vi "Measurement Logic.vi"(8 "error in":errorcluster, 9 "measurement configuration":T2={"Automation Test"=FALSE, "Power sequencing file path"="", "RFmxVNA name"="5842_0", "vCal Name"="VNA-5633", "RFmxVNA Calset Enable"=FALSE, "RFmxVNA Calset Interpolation"=FALSE, "Calset File Path (String)"="", "RFmxVNA attenuation mode"=enum."s2p File", "RFmxVNA Port1 s2p file path (String)"="", "RFmxVNA Port1 s-parameters orientation"=enum."Port2 Towards DUT", "RFmxVNA Port1 Power Compensation"=FALSE, "RFmxVNA Port2 s2p file path (String)"="", "RFmxVNA Port2 s-parameters orientation"=enum."Port1 Towards DUT", "RFmxVNA Port2 Power Compensation"=FALSE, "Port1 Power Level (dBm)"=2.0, "Port1 Test Receiver Attenuation (dB)"=1.2, "Port2 Power Level (dBm)"=2.0, "Port2 Test Receiver Attenuation (dB)"=1.2, "IF Bandwidth (Hz)"=1.0, "Action"=enum."Measure", "Pulse Mode Enabled"=FALSE, "Pulse Period"=0.001, "Pulse Modulator Delay"=0.0, "Pulse Modulator Width"=0.0001, "Pulse Acquisition Auto"=FALSE, "Pulse Acquisition Delay"=2e-05, "Pulse Acquisition Width"=4.665e-05, "Start Frequency (Hz)"=4000000000.0, "Stop Frequency (Hz)"=26000000000.0, "Number of Points"=200, "Measurement S-Parameters"=["S11", "S12", "S21", "S22"], "Phase Trace Type"=0, "Magnitude Units"=0, "SnP File Path (String)"="", "Averaging Enabled"=FALSE, "Averaging Count"=0, "Power sequencing file validity check"=TRUE} {"Magnitude Units" items=["dB", "Linear"]; "Phase Trace Type" items=["Wrapped", "Unwrapped"]; "Stop Frequency (Hz)" format="%.3p"; "Start Frequency (Hz)" format="%.3p"; "Pulse Acquisition Width" format="%.2p"; "Pulse Acquisition Delay" format="%.2p"; "Pulse Modulator Width" format="%.2p"; "Pulse Modulator Delay" format="%.2p"; "Pulse Period" format="%.2p"; "IF Bandwidth (Hz)" format="%.2p"; "Port2 Test Receiver Attenuation (dB)" format="%.2f"; "Port2 Power Level (dBm)" format="%.2f"; "Port1 Test Receiver Attenuation (dB)" format="%.2f"; "Port1 Power Level (dBm)" format="%.2f"}, 10 "measure call context in":refnum<class "Measure Call Context.lvclass">) -> (0 "error out":errorcluster, 1 "measurement results":T1, 2 "measure call context out":refnum<class "Measure Call Context.lvclass">)   [LabVIEW 2023, in "FPT_SParam.lvclass"]
doc: "Contains the core logic for executing the measurement."
uses:
  FPT_SParam.lvclass
  FPT_SParam.lvclass/FPT_SParam.ctl
  Measurement Configuration.ctl
  Measurement Results.ctl
  <vilib>/Analysis/NI_AALBase.lvlib
  <vilib>/Analysis/baseanly.llb/Mean (DBL).vi
  <vilib>/Plug-In SDKs/Measurements/Measure Call Context/Measure Call Context.lvclass
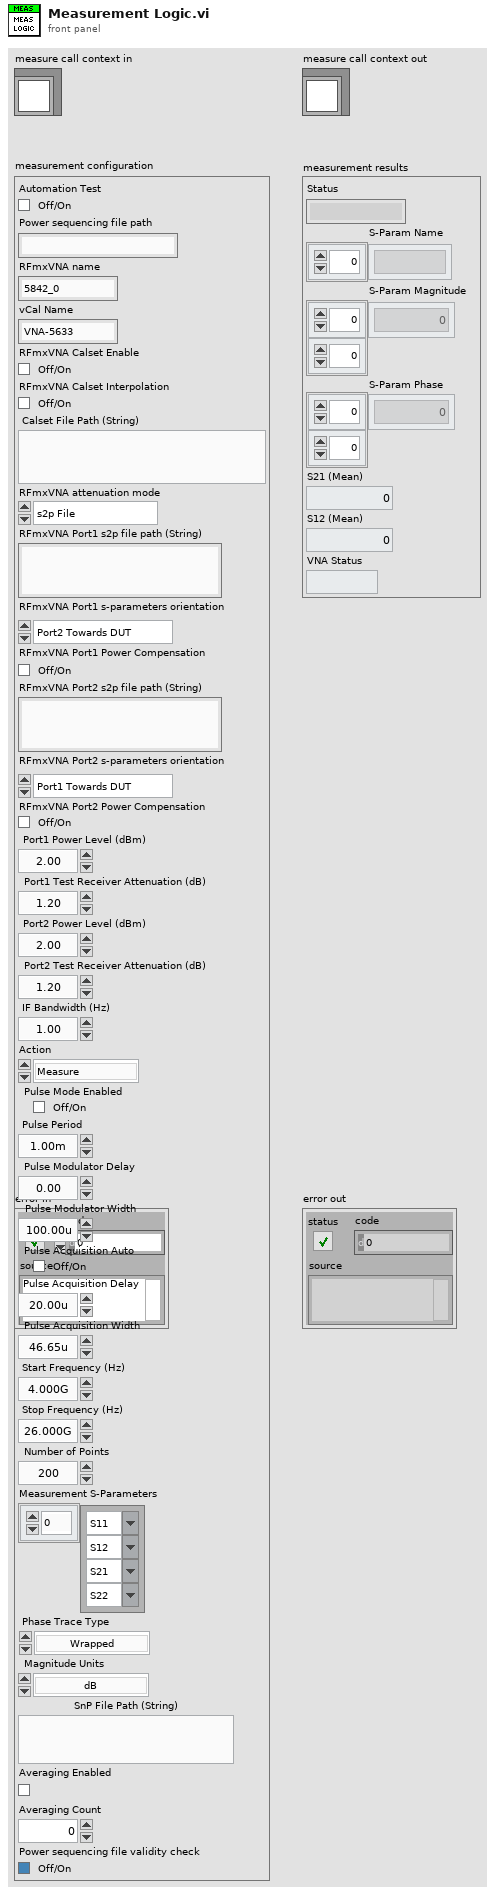
[diagram p1: front panel]
types:
  T1 = typedef "FPT_SParam.lvclass/Measurement Results.ctl" = cluster{"Status":string, "S-Param Name":string[], "S-Param Magnitude":dbl[][], "S-Param Phase":dbl[][], "S21 (Mean)":dbl, "S12 (Mean)":dbl, "VNA Status":string}
  T2 = typedef "FPT_SParam.lvclass/Measurement Configuration.ctl" = cluster{"Automation Test":bool, "Power sequencing file path":string, "RFmxVNA name":string, "vCal Name":string, "RFmxVNA Calset Enable":bool, "RFmxVNA Calset Interpolation":bool, "Calset File Path (String)":string, "RFmxVNA attenuation mode":enum32{"<None>", "s2p File"}, "RFmxVNA Port1 s2p file path (String)":string, "RFmxVNA Port1 s-parameters orientation":enum32{"Port1 Towards DUT", "Port2 Towards DUT"}, "RFmxVNA Port1 Power Compensation":bool, "RFmxVNA Port2 s2p file path (String)":string, "RFmxVNA Port2 s-parameters orientation":enum32{"Port1 Towards DUT", "Port2 Towards DUT"}, "RFmxVNA Port2 Power Compensation":bool, "Port1 Power Level (dBm)":dbl, "Port1 Test Receiver Attenuation (dB)":dbl, "Port2 Power Level (dBm)":dbl, "Port2 Test Receiver Attenuation (dB)":dbl, "IF Bandwidth (Hz)":dbl, "Action":enum32{"Calibrate", "Measure"}, "Pulse Mode Enabled":bool, "Pulse Period":dbl, "Pulse Modulator Delay":dbl, "Pulse Modulator Width":dbl, "Pulse Acquisition Auto":bool, "Pulse Acquisition Delay":dbl, "Pulse Acquisition Width":dbl, "Start Frequency (Hz)":dbl, "Stop Frequency (Hz)":dbl, "Number of Points":i32, "Measurement S-Parameters":string[], "Phase Trace Type":i32, "Magnitude Units":i32, "SnP File Path (String)":string, "Averaging Enabled":bool, "Averaging Count":u32, "Power sequencing file validity check":bool}
  T3 = cluster{"measurement configuration":T2, "measurement results":T1, "CustomData":cluster{"Valid CSV":bool}}
  T4 = enum32{"Power On Dut", "Switching", "De-embedding + Measurement", "Power Off Dut"}[]
  T5 = typedef "RFmxVNA Config - SParam.ctl" = cluster{"Resource Name":refnum<k15>, "vCal Name":string, "RFmxVNA Calset Enable":bool, "RFmxVNA Calset Interpolation":bool, "Calset File Path":string, "RFmxVNA attenuation mode":enum32{"<None>", "s2p File"}, "RFmxVNA Port1 s2p file path":string, "RFmxVNA Port1 s-parameters orientation":enum32{"Port1 Towards DUT", "Port2 Towards DUT"}, "RFmxVNA Port1 Power Compensation":bool, "RFmxVNA Port2 s2p file path":string, "RFmxVNA Port2 s-parameters orientation":enum32{"Port1 Towards DUT", "Port2 Towards DUT"}, "RFmxVNA Port2 Power Compensation":bool, "Port1 Power Level (dBm)":dbl, "Port1 Test Receiver Attenuation (dB)":dbl, "Port2 Power Level (dBm)":dbl, "Port2 Test Receiver Attenuation (dB)":dbl, "IF Bandwidth (Hz)":dbl, "Frequency Sweep":cluster{"Start Frequency (Hz)":dbl, "Stop Frequency (Hz)":dbl, "Number of Points":i32}}
  T6 = typedef "Test Config - SParam.ctl" = cluster{"Action":enum16{"Calibrate", "Measure"}, "Pulse Mode":cluster{"Pulse Mode Enabled":bool, "Pulse Period (s)":dbl, "Pulse Modulator Delay (s)":dbl, "Pulse Modulator Width (s)":dbl, "Pulse Acquisition Auto":bool, "Pulse Acquisition Delay (s)":dbl, "Pulse Acquisition Width (s)":dbl}, "Frequency Sweep":cluster{"Start Frequency (Hz)":dbl, "Stop Frequency (Hz)":dbl, "Number of Points":i32}, "S-Parameters":string[], "Magnitude Units":i32, "Phase Trace Type":i32, "SnP File Path":string, "Averaging Enabled":bool, "Averaging Count":u32}
  T7 = typedef "Event Messenger-bool.lvlib/))Channel.ctl" = refnum<queue>
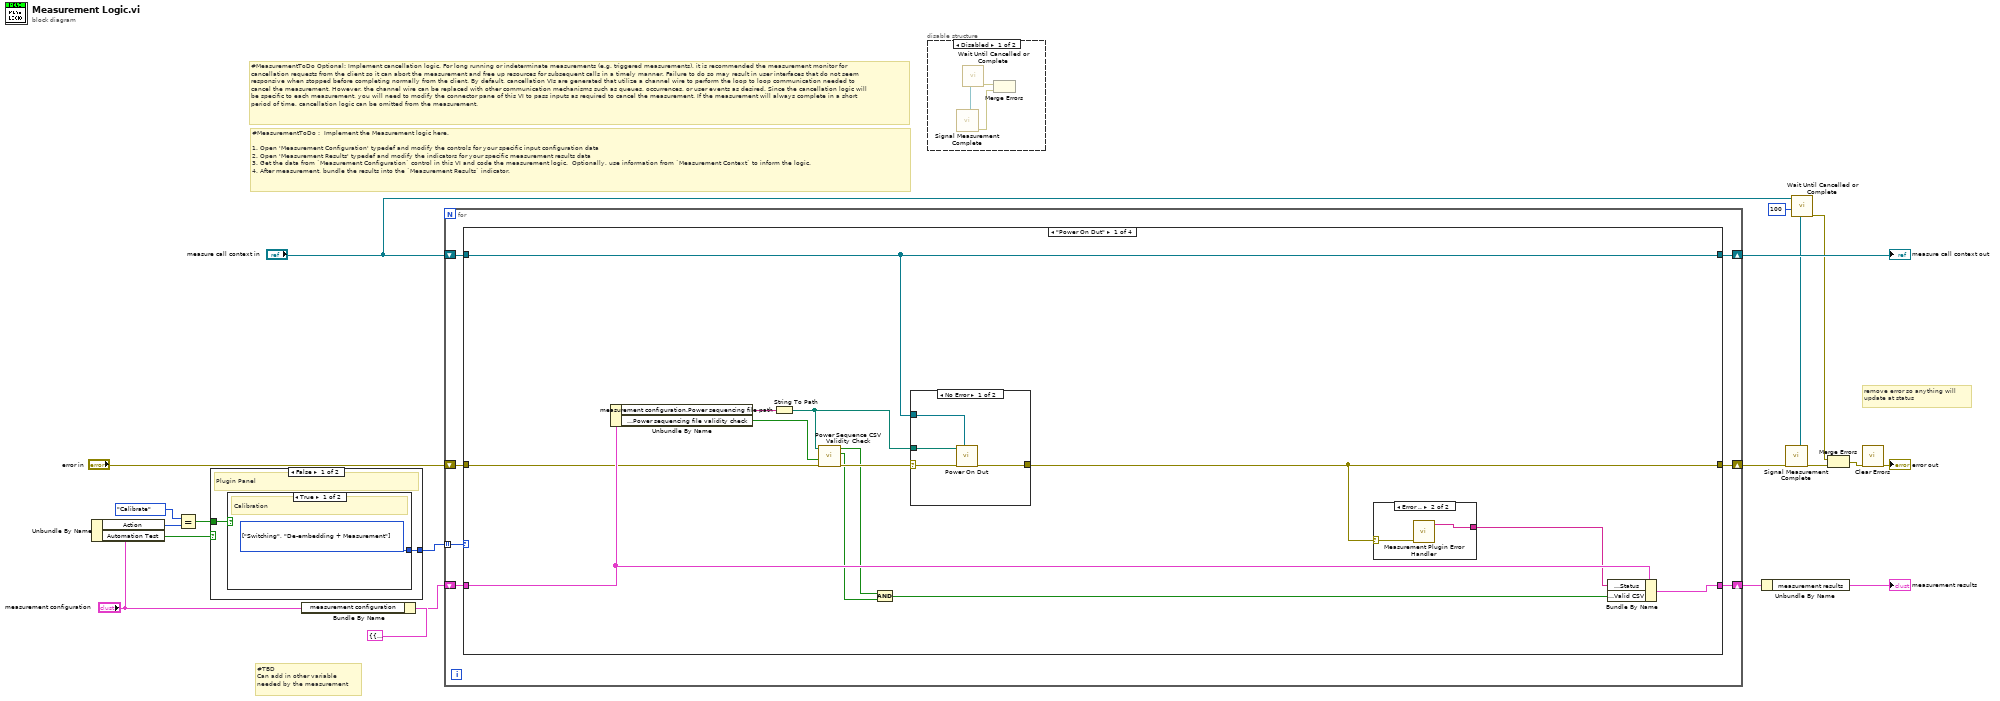
[diagram p0: block diagram]
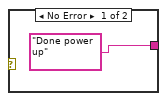
[diagram p3: hidden frame]
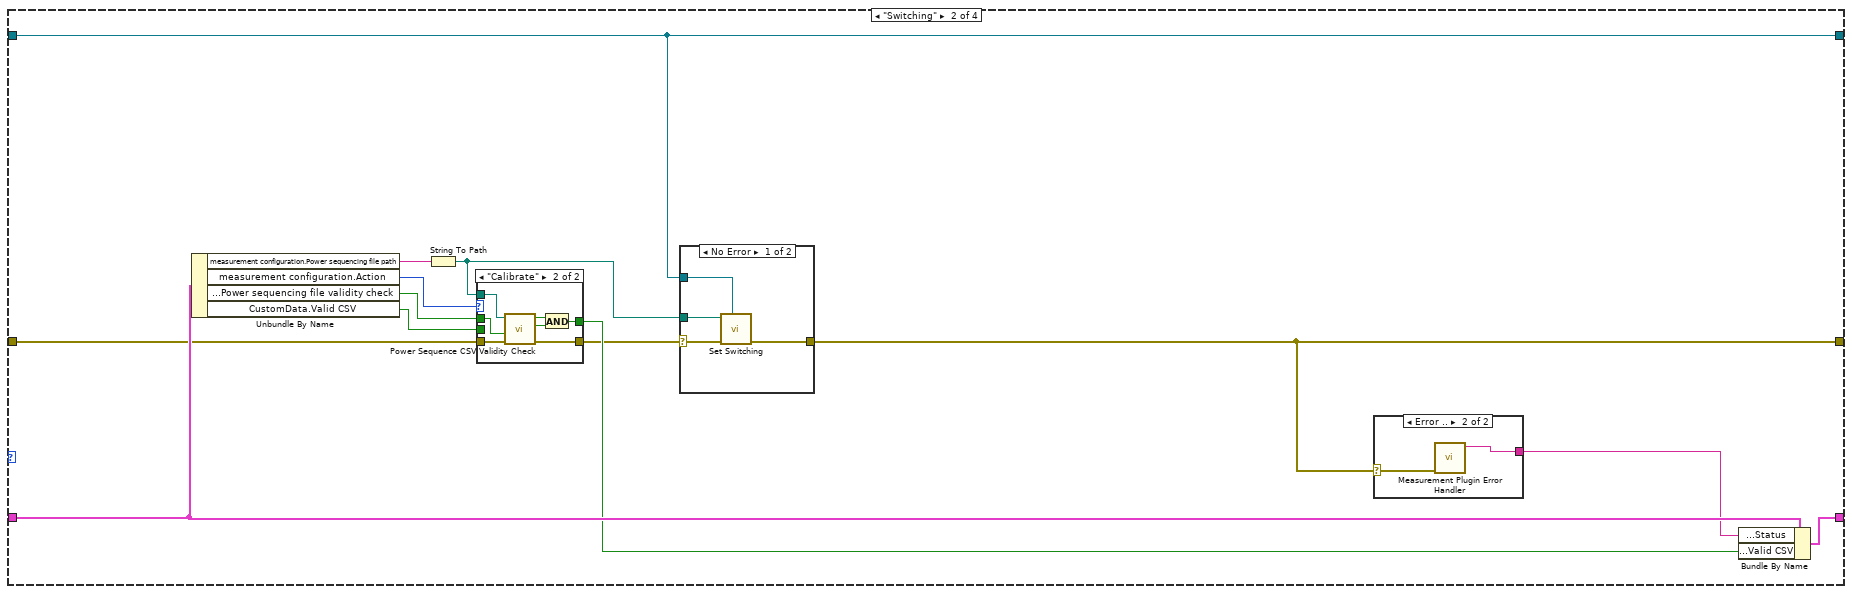
[diagram p4: hidden frame]
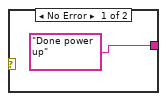
[diagram p7: hidden frame]
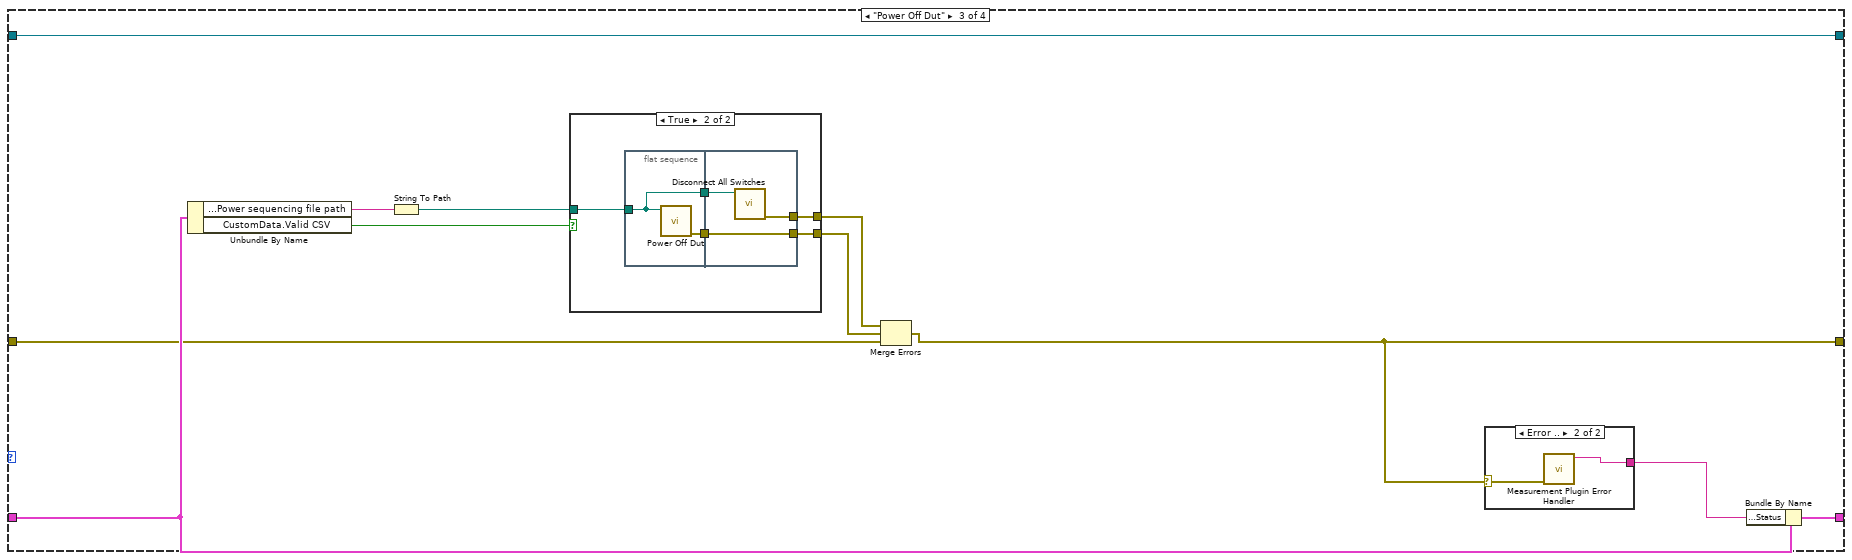
[diagram p8: hidden frame]
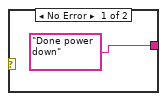
[diagram p10: hidden frame]
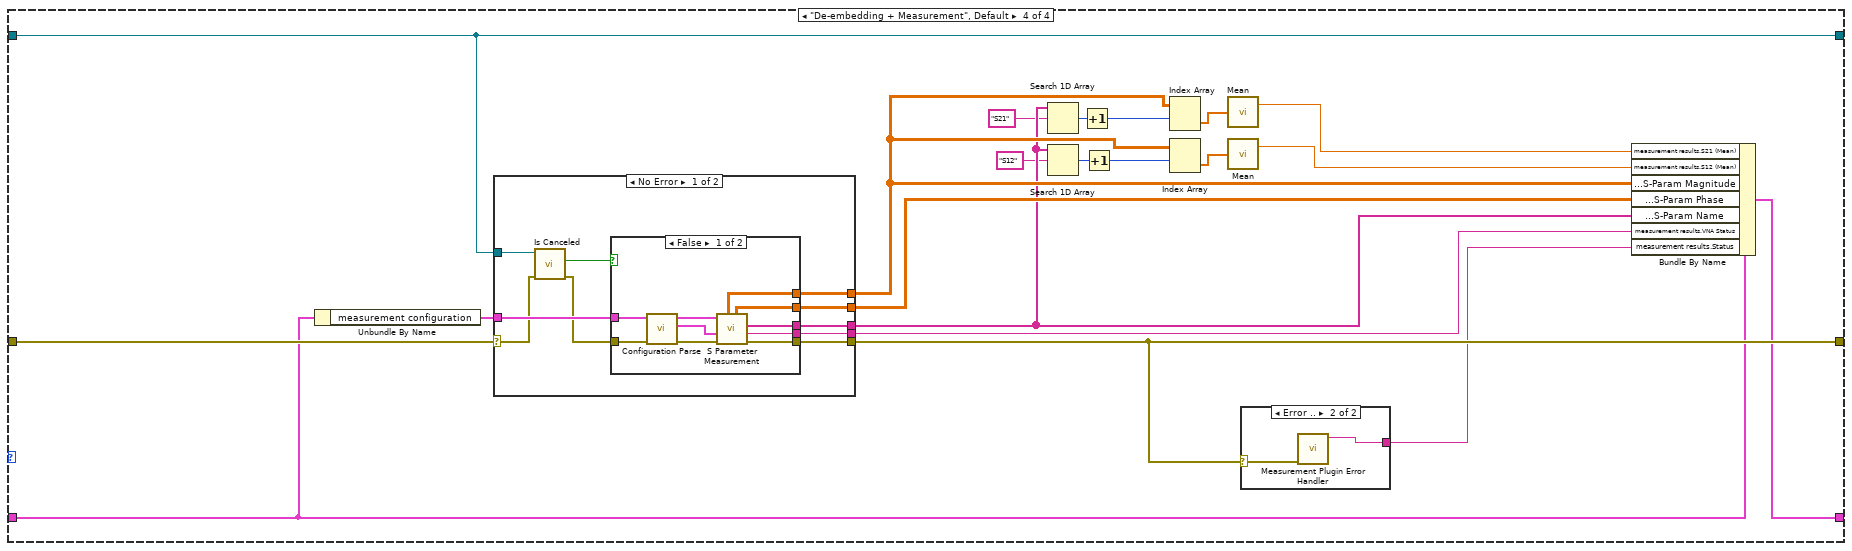
[diagram p11: hidden frame]
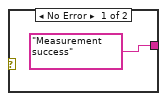
[diagram p12: hidden frame]
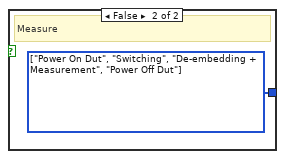
[diagram p16: hidden frame]
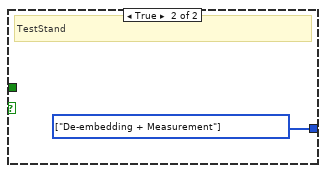
[diagram p17: hidden frame]
diagram:
  # "remove error so anything will\nupdate at status"
  # "#TBD\nCan add in other variable\nneeded by the measurement"
  # "#MeasurementToDo Optional: Implement cancellation logic. For long running or indeterminate measurements (e.g. triggered measurements), it is recommended the measurement monitor for cancellation requests from the client so it can abort the measurement and free up resources for subsequent calls in a timely manner. Failure to do so may result in user interfaces that do not seem responsive when stopped before completing normally from the client. By default, cancellation VIs are generated that utilize a channel wire to perform the loop to loop communication needed to cancel the measurement. However, the channel wire can be replaced with other communication mechanisms such as queues, occurrences, or user events as desired. Since the cancellation logic will be specific to each measurement, you will need to modify the connector pane of this VI to pass inputs as required to cancel the measurement. If the measurement will always complete in a short period of time, cancellation logic can be omitted from the measurement."
  # "#MeasurementToDo :  Implement the Measurement logic here.\n\n1. Open 'Measurement Configuration' typedef and modify the controls for your specific input configuration data\n2. Open 'Measurement Results' typedef and modify the indicators for your specific measurement results data\n3. Get the data from `Measurement Configuration` control in this VI and code the measurement logic.  Optionally, use information from `Measurement Context` to inform the logic.\n4. After measurement, bundle the results into the `Measurement Results` indicator."
  n1 = Unbundle By Name("measurement configuration") -> ("Action"=w12:enum32{"Calibrate", "Measure"}, "Automation Test"=w9:bool)
  n2 = Equal?(x=enum32{"Calibrate", "Measure"}."Calibrate", y=w12) -> (x = y?=w8:bool)
  n3 = case shown="False" w9 {
    tunnel: [w22 w25] -> w10
    tunnel: w8 -> [w21 _]
    frame False {
      # "Plugin Panel"
      n4 = case shown="True" w21 {
        tunnel: [w23 w24] -> w22
        frame True {
          w23 = T4 [enum."Switching", enum."De-embedding + Measurement"] items=["Power On Dut", "Switching", "De-embedding + Measurement", "Power Off Dut"]
          # "Calibration"
        }
        frame False {
          w24 = T4 [enum."Power On Dut", enum."Switching", enum."De-embedding + Measurement", enum."Power Off Dut"] items=["Power On Dut", "Switching", "De-embedding + Measurement", "Power Off Dut"]
          # "Measure"
        }
      }
    }
    frame True {
      w25 = T4 [enum."De-embedding + Measurement"] items=["Power On Dut", "Switching", "De-embedding + Measurement", "Power Off Dut"]
      # "TestStand"
    }
  }
  n5 = Bundle By Name(cluster=T3 {"measurement configuration"={"Automation Test"=FALSE, "Power sequencing file path"="", "RFmxVNA name"="5842_0", "vCal Name"="VNA-5633", "RFmxVNA Calset Enable"=FALSE, "RFmxVNA Calset Interpolation"=FALSE, "Calset File Path (String)"="", "RFmxVNA attenuation mode"=enum."s2p File", "RFmxVNA Port1 s2p file path (String)"="", "RFmxVNA Port1 s-parameters orientation"=enum."Port2 Towards DUT", "RFmxVNA Port1 Power Compensation"=FALSE, "RFmxVNA Port2 s2p file path (String)"="", "RFmxVNA Port2 s-parameters orientation"=enum."Port1 Towards DUT", "RFmxVNA Port2 Power Compensation"=FALSE, "Port1 Power Level (dBm)"=2.0, "Port1 Test Receiver Attenuation (dB)"=1.2, "Port2 Power Level (dBm)"=2.0, "Port2 Test Receiver Attenuation (dB)"=1.2, "IF Bandwidth (Hz)"=1.0, "Action"=enum."Measure", "Pulse Mode Enabled"=FALSE, "Pulse Period"=0.001, "Pulse Modulator Delay"=0.0, "Pulse Modulator Width"=0.0001, "Pulse Acquisition Auto"=FALSE, "Pulse Acquisition Delay"=2e-05, "Pulse Acquisition Width"=4.665e-05, "Start Frequency (Hz)"=4000000000.0, "Stop Frequency (Hz)"=26000000000.0, "Number of Points"=200, "Measurement S-Parameters"=["S11", "S12", "S21", "S22"], "Phase Trace Type"=0, "Magnitude Units"=0, "SnP File Path (String)"="", "Averaging Enabled"=FALSE, "Averaging Count"=0, "Power sequencing file validity check"=TRUE}, "measurement results"={"Status"="", "S-Param Name"=[], "S-Param Magnitude"=[], "S-Param Phase"=[], "S21 (Mean)"=0.0, "S12 (Mean)"=0.0, "VNA Status"=""}, "CustomData"={"Valid CSV"=FALSE}}, "measurement configuration"="measurement configuration") -> (w18:T3)
  n6 = for {
    tunnel: w10 -> [w31] mode=indexing
    shift-right: [w26] -> w4
    shift-left: "error in" -> [w32]
    shift-right: [w27] -> w16
    shift-left: w18 -> [w30]
    shift-right: [w28] -> w17
    shift-left: "measure call context in" -> [w29]
    n7 = case shown="\"Power On Dut\"" w31 {
      tunnel: w32 -> [w39 w59 w89 w123]
      tunnel: w30 -> [w45 w66 w90 w122]
      tunnel: w29 -> [w40 w61 w93 w109]
      tunnel: [w41 w62 w88 w128] -> w26
      tunnel: [w40 w61 w93 w109] -> w28
      tunnel: [w43 w64 w91 w126] -> w27
      frame "Power On Dut" {
        n8 = Unbundle By Name(w45) -> ("measurement configuration.Power sequencing file path"=w42:string, "measurement configuration.Power sequencing file validity check"=w38:bool)
        n9 = String To Path(string=w42) -> (path=w37:path)
        n10 = call "Power Sequence CSV Validity Check.vi"("error in"=w39, "Enable Validity Check?"=w38, "File Path"=w37) -> ("error out"=w36:errorcluster, "Valid Execution Order"=w34:bool, "All Instruments Available"=w35:bool)  [unwired: 5 in, 1 out]
        n11 = And(x=w35, y=w34) -> (x .and. y?=w33:bool)
        n12 = case shown="No Error" w36 {
          selector: w36 -> [w46 w50]
          tunnel: w37 -> [w49 _]
          tunnel: [w48 w50] -> w41
          tunnel: w40 -> [w47 _]
          frame No Error {
            n13 = call "Power On Dut.vi"("measure call context in"=w47, "error in"=w46, "Power sequencing file path"=w49) -> ("error out"=w48:errorcluster)  [unwired: 7 in, 1 out]
          }
          frame Error {
          }
        }
        n14 = case shown="Error .." w41 {
          selector: w41 -> [_ w53]
          tunnel: ["Done power up" w52] -> w44
          frame No Error {
          }
          frame Error {
            n15 = call "Measurement Plugin Error Handler.vi"("error in"=w53) -> ("Status Message (Error)"=w52:string)  [unwired: 9 in, 1 out]
          }
        }
        n16 = Bundle By Name(cluster=w45, "measurement results.Status"=w44, "CustomData.Valid CSV"=w33) -> (w43:T3)
      }
      frame "Switching" {
        n17 = Unbundle By Name(w66) -> ("measurement configuration.Power sequencing file path"=w63:string, "measurement configuration.Action"=w60:enum32{"Calibrate", "Measure"}, "measurement configuration.Power sequencing file validity check"=w57:bool, "CustomData.Valid CSV"=w56:bool)
        n18 = String To Path(string=w63) -> (path=w58:path)
        n19 = case shown="\"Calibrate\"" w60 {
          tunnel: w59 -> [w68 w75]
          tunnel: [w68 w74] -> w54
          tunnel: [w67 w71] -> w55
          tunnel: w58 -> [_ w70]
          tunnel: w57 -> [_ w69]
          tunnel: w56 -> [w67 _]
          frame Default {
          }
          frame "Calibrate" {
            n20 = call "Power Sequence CSV Validity Check.vi"("error in"=w75, "Enable Validity Check?"=w69, "File Path"=w70) -> ("error out"=w74:errorcluster, "Valid Execution Order"=w72:bool, "All Instruments Available"=w73:bool)  [unwired: 5 in, 1 out]
            n21 = And(x=w73, y=w72) -> (x .and. y?=w71:bool)
          }
        }
        n22 = case shown="No Error" w54 {
          selector: w54 -> [w76 w80]
          tunnel: [w79 w80] -> w62
          tunnel: w58 -> [w78 _]
          tunnel: w61 -> [w77 _]
          frame No Error {
            n23 = call "Set Switching.vi"("measure call context in"=w77, "error in"=w76, "File Path"=w78) -> ("error out"=w79:errorcluster)  [unwired: 7 in, 1 out]
          }
          frame Error {
          }
        }
        n24 = case shown="Error .." w62 {
          selector: w62 -> [_ w83]
          tunnel: ["Done power up" w82] -> w65
          frame No Error {
          }
          frame Error {
            n25 = call "Measurement Plugin Error Handler.vi"("error in"=w83) -> ("Status Message (Error)"=w82:string)  [unwired: 9 in, 1 out]
          }
        }
        n26 = Bundle By Name(cluster=w66, "measurement results.Status"=w65, "CustomData.Valid CSV"=w55) -> (w64:T3)
      }
      frame "Power Off Dut" {
        n27 = Unbundle By Name(w90) -> ("measurement configuration.Power sequencing file path"=w94:string, "CustomData.Valid CSV"=w84:bool)
        n28 = String To Path(string=w94) -> (path=w87:path)
        n29 = case shown="True" w84 {
          tunnel: w87 -> [_ w97]
          tunnel: [_ w96] -> w86
          tunnel: [_ w95] -> w85
          frame False {
          }
          frame True {
            n30 = flat-sequence {
              tunnel: w97 -> [w100]
              tunnel: [w101] -> w99
              tunnel: [w100] -> w98
              tunnel: [w104] -> w96
              tunnel: w99 -> [w104]
              tunnel: [w103] -> w95
              tunnel: w98 -> [w102]
              frame #0 {
                n31 = call "Power Off Dut.vi"("Power Sequencing File Path"=w100) -> ("error out"=w101:errorcluster)  [unwired: 10 in]
              }
              frame #1 {
                n32 = call "Disconnect All Switches.vi"("File Path"=w102) -> ("error out"=w103:errorcluster)  [unwired: 10 in]
              }
            }
          }
        }
        n33 = Merge Errors(w85, w86, w89) -> (w88:errorcluster)
        n34 = case shown="Error .." w88 {
          selector: w88 -> [_ w107]
          tunnel: ["Done power down" w106] -> w92
          frame No Error {
          }
          frame Error {
            n35 = call "Measurement Plugin Error Handler.vi"("error in"=w107) -> ("Status Message (Error)"=w106:string)  [unwired: 9 in, 1 out]
          }
        }
        n36 = Bundle By Name(cluster=w90, "measurement results.Status"=w92) -> (w91:T3)
      }
      frame "De-embedding + Measurement", Default {
        n37 = Unbundle By Name(w122) -> ("measurement configuration"=w108:T2)
        n38 = case shown="No Error" w123 {
          selector: w123 -> [w135 w153]
          tunnel: [w141 w153] -> w128
          tunnel: [w140 _] -> w117
          tunnel: [w139 _] -> w125
          tunnel: [w138 _] -> w124
          tunnel: [w137 _] -> w116
          tunnel: w108 -> [w136 _]
          tunnel: w109 -> [w132 _]
          frame No Error {
            n39 = call <vilib>:"Is Canceled.vi"("error in"=w135, "measure call context in"=w132) -> ("error out"=w134:errorcluster, "is canceled?"=w133:bool)  [unwired: 7 in, 1 out]
            n40 = case shown="False" w133 {
              tunnel: [w151 w152] -> w141
              tunnel: [w147 _] -> w140
              tunnel: [w146 _] -> w139
              tunnel: [w145 _] -> w138
              tunnel: [w144 _] -> w137
              tunnel: w136 -> [w143 _]
              tunnel: w134 -> [w142 w152]
              frame False {
                n41 = call "Configuration Parse.vi"("error in"=w142, "Measurement Configuration"=w143) -> ("error out"=w149:errorcluster, "RFmxVNA Settings"=w150:T5, "Test Configuration"=w148:T6)  [unwired: 7 in]
                n42 = call "S Parameter Measurement.vi"("error in"=w149, "RFmxVNA Settings"=w150, "Test Configuration"=w148) -> ("error out"=w151:errorcluster, "VNA Status"=w145:string, "S-Param Name"=w144:string[], "S-Param Phase"=w146:dbl[][], "S-Param Magnitude"=w147:dbl[][])  [unwired: 3 in, 1 out]
              }
              frame True {
              }
            }
          }
          frame Error {
          }
        }
        n43 = Search 1D Array(1D array=w116, element="S21") -> (index of element=w113:i32)  [unwired: 1 in]
        n44 = Search 1D Array(1D array=w116, element="S12") -> (index of element=w111:i32)  [unwired: 1 in]
        n45 = Increment(x=w113) -> (x+1=w112:i32)
        n46 = Increment(x=w111) -> (x+1=w110:i32)
        n47 = Index Array(array=w117, index (row)=w112) -> (element=w121:dbl[])  [unwired: 1 in]
        n48 = Index Array(array=w117, index (row)=w110) -> (element=w119:dbl[])  [unwired: 1 in]
        n49 = call-poly <vilib>:"Mean.vi"("X"=w121) -> ("mean"=w120:dbl)  [unwired: 1 out]
        n50 = call-poly <vilib>:"Mean.vi"("X"=w119) -> ("mean"=w118:dbl)  [unwired: 1 out]
        n51 = case shown="Error .." w128 {
          selector: w128 -> [_ w131]
          tunnel: ["Measurement success" w130] -> w127
          frame No Error {
          }
          frame Error {
            n52 = call "Measurement Plugin Error Handler.vi"("error in"=w131) -> ("Status Message (Error)"=w130:string)  [unwired: 9 in, 1 out]
          }
        }
        n53 = Bundle By Name(cluster=w122, "measurement results.S21 (Mean)"=w120, "measurement results.S12 (Mean)"=w118, "measurement results.S-Param Magnitude"=w117, "measurement results.S-Param Phase"=w125, "measurement results.S-Param Name"=w116, "measurement results.VNA Status"=w124, "measurement results.Status"=w127) -> (w126:T3)
      }
    }
  }
  "measure call context out" <- w17
  n54 = disable-structure shown="Disabled" {
    frame Disabled {
      n55 = call "Signal Measurement Complete.vi"() -> ("error out"=w155:errorcluster, "done channel"=w156:T7)  [unwired: 10 in]
      n56 = call "Wait Until Cancelled or Complete.vi"("done channel"=w156) -> ("error out"=w154:errorcluster)  [unwired: 9 in, 1 out]
      n57 = Merge Errors(w154, w155) -> ()  [unwired: 1 out]
    }
    frame Enabled {
    }
  }
  n58 = Unbundle By Name(w16) -> ("measurement results"=→"measurement results":T1)
  n59 = call "Signal Measurement Complete.vi"("error in (no error)"=w4) -> ("error out"=w3:errorcluster, "done channel"=w2:T7)  [unwired: 9 in]
  n60 = call "Wait Until Cancelled or Complete.vi"("done channel"=w2, "ms polling interval"=100, "measure call context in"="measure call context in") -> ("error out"=w6:errorcluster)  [unwired: 7 in, 1 out]
  n61 = Merge Errors(w6, w3) -> (w7:errorcluster)
  n62 = call <vilib>:"Clear Errors.vi"("error in (no error)"=w7) -> ("error out"=→"error out":errorcluster)  [unwired: 5 in, 1 out]
